vi "login_TCT.vi"() -> (1 "LOGIN":bool=TRUE, 3 "Login String":string=" has Successfully Logged in since :: 17:01:04")   [LabVIEW 2026]
uses:
  <vilib>/Utility/file.llb/Read Delimited Spreadsheet (string).vi
panel:
  in  "Cancel Button":bool
  in  "Log In Button":bool
  out "Login ok":bool=TRUE
  in  "PASSWORD":string
  in  "USER NAME":string
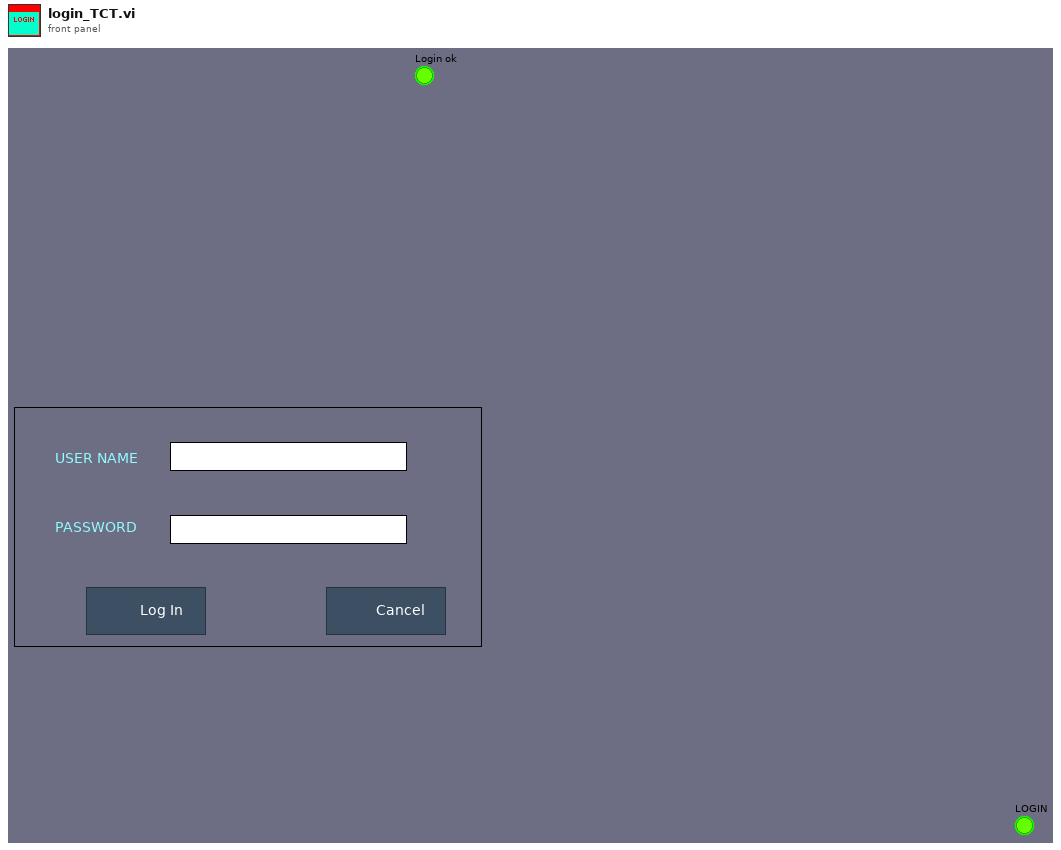
[diagram p1: front panel]
types:
  T1 = enum16{"open", "replace", "create", "open or create", "replace or create", "replace or create with confirmation"}
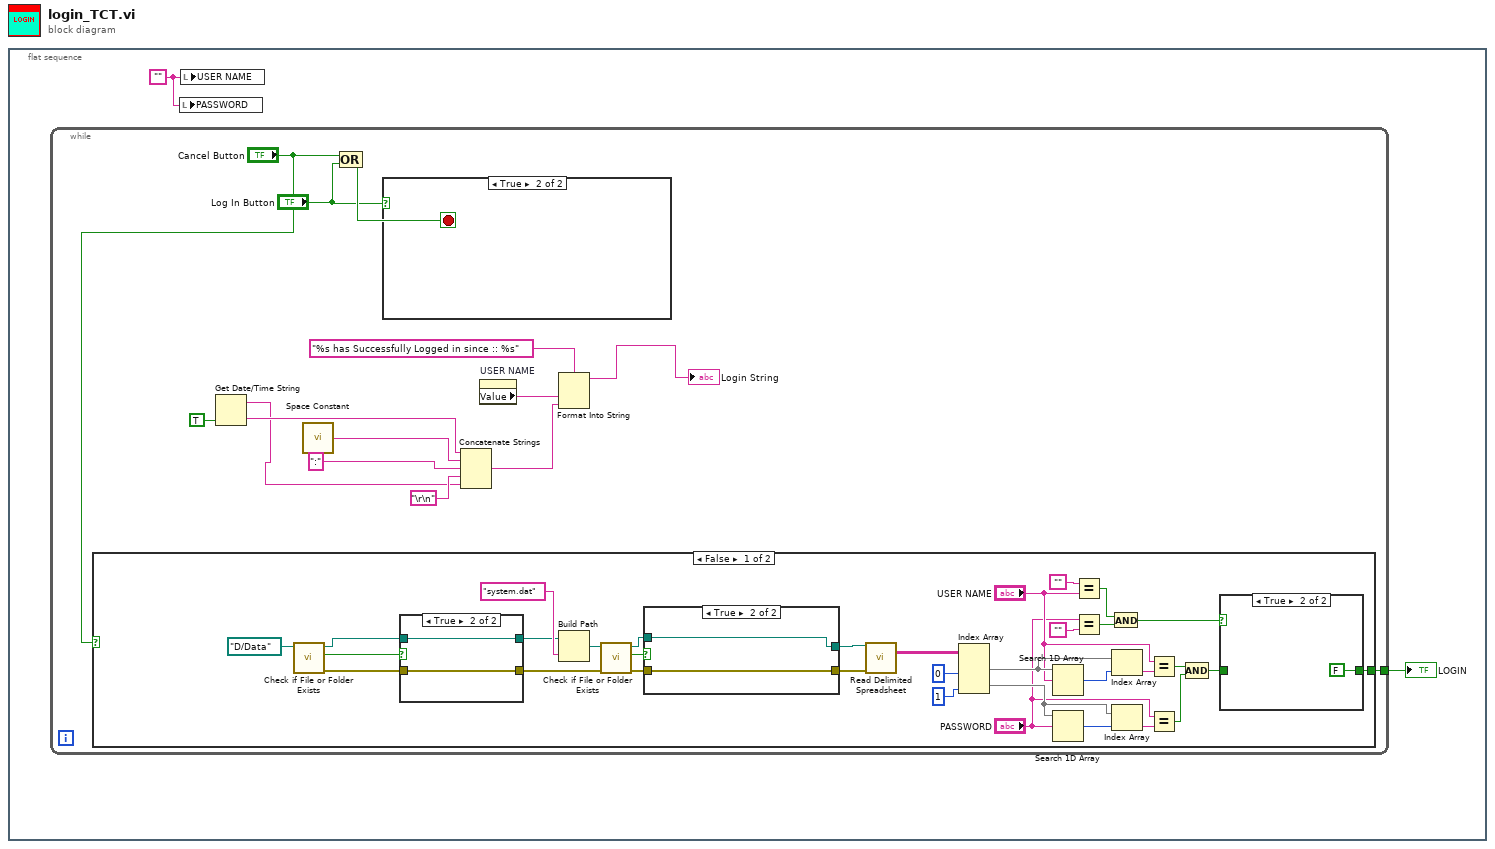
[diagram p0: block diagram]
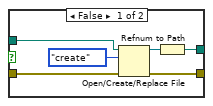
[diagram p2: hidden frame]
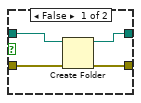
[diagram p3: hidden frame]
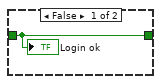
[diagram p4: hidden frame]
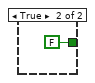
[diagram p5: hidden frame]
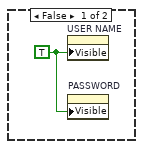
[diagram p6: hidden frame]
diagram:
  n1 = flat-sequence {
    frame #0 {
      w1 = ""
      n2 = while {
        tunnel: [w12] -> w2
        stop <- w14 stop-if-true
        n3 = case shown="False" "Cancel Button" {
          tunnel: [w26 FALSE] -> w12
          frame False {
            n4 = call <vilib>:"Check if File or Folder Exists.vi"("path"=path "D:/Data" ("file path (dialog if empty)")) -> ("error out"=w23:errorcluster, "file or folder exists?"=w18:bool, "dup path"=w37:path)  [unwired: 8 in]
            n5 = case shown="True" w18 {
              tunnel: w37 -> [w61 w62]
              tunnel: [w60 w62] -> w24
              tunnel: w23 -> [w59 w63]
              tunnel: [w58 w63] -> w22
              frame False {
                n6 = Create Folder(path (use dialog)=w61, error in=w59) -> (created path=w60:path, error out=w58:errorcluster)  [unwired: 1 in, 1 out]
              }
              frame True {
              }
            }
            n7 = Build Path(base path=w24, name or relative path="system.dat") -> (appended path=w20:path)
            n8 = call <vilib>:"Check if File or Folder Exists.vi"("error in (no error)"=w22, "path"=w20) -> ("error out"=w21:errorcluster, "file or folder exists?"=w17:bool, "dup path"=w19:path)  [unwired: 7 in]
            n9 = case shown="True" w17 {
              tunnel: [w55 w56] -> w36
              tunnel: [w54 w57] -> w35
              tunnel: w19 -> [w50 w57]
              tunnel: w21 -> [w51 w56]
              frame False {
                n10 = Open/Create/Replace File(file path (use dialog)=w50, error in=w51, operation (0:open)=T1."create") -> (refnum out=w53:refnum<file>, error out=w55:errorcluster)  [unwired: 3 in, 1 out]
                n11 = Refnum to Path(1:w53) -> (0:w54:path)
              }
              frame True {
              }
            }
            n12 = call-poly <vilib>:"Read Delimited Spreadsheet.vi"("file path (dialog if empty)"=w35, "error in (no error)"=w36) -> ("all rows"=w39:string[][])  [unwired: 8 in, 5 out]
            n13 = Index Array "Index Array"(array=w39, index (col) #1=0 ("disabled index (col)"), index (col) #2=1 ("index (col)")) -> (element #1=w42:string[], element #2=w43:string[])  [unwired: 2 in]
            n14 = Search 1D Array(1D array=w42, element="USER NAME") -> (index of element=w47:i32)  [unwired: 1 in]
            n15 = Search 1D Array(1D array=w43, element="PASSWORD") -> (index of element=w48:i32)  [unwired: 1 in]
            n16 = Equal?(x="", y="USER NAME") -> (x = y?=w29:bool)
            n17 = Equal?(x="PASSWORD", y="") -> (x = y?=w30:bool)
            n18 = And(x=w29, y=w30) -> (x .and. y?=w27:bool)
            n19 = Index Array(array=w42, index=w47) -> (element=w49:string)
            n20 = Index Array(array=w43, index=w48) -> (element=w46:string)
            n21 = Equal?(x="USER NAME", y=w49) -> (x = y?=w44:bool)
            n22 = Equal?(x="PASSWORD", y=w46) -> (x = y?=w45:bool)
            n23 = Compound Arithmetic op=AND(w44, w45) -> (w28:bool)
            n24 = case shown="True" w27 {
              tunnel: w28 -> [w64 _]
              tunnel: [w64 FALSE] -> w26
              frame False {
                "Login ok" <- w64
              }
              frame True {
              }
            }
          }
          frame True {
          }
        }
        n25 = Get Date/Time String(want seconds? (F)=TRUE) -> (date string=w3:string, time string=w9:string)  [unwired: 2 in]
        n26 = call <vilib>:"Space Constant.vi"() -> ("String"=w11:string)
        n27 = Compound Arithmetic op=OR("Cancel Button", "Log In Button") -> (w14:bool)
        n28 = case shown="True" "Log In Button" {
          frame False {
            w67 = TRUE
            n29 = property on="USER NAME" class="Str"("Visible"=w67) -> ()  [unwired: 2 in, 2 out]
            n30 = property on="PASSWORD" class="Str"("Visible"=w67) -> ()  [unwired: 2 in, 2 out]
          }
          frame True {
          }
        }
        n31 = Concatenate Strings(w9, w11, ":" ("string"), "\r\n", w3) -> (w10:string)
        n32 = property on="USER NAME" class="Str"() -> ("Value"=w15:string)  [unwired: 2 in, 2 out]
        n33 = Format Into String(format string="%s has Successfully Logged in since :: %s", w15, w10) -> (resulting string=→"Login String":string)  [unwired: 2 in, 1 out]
      }
      "LOGIN" <- w2
      n34 = local write "PASSWORD"(w1) -> ()
      n35 = local write "USER NAME"(w1) -> ()
    }
  }
